vi "FuncVI-MSE.vi"(5 "InstanceRef":T2, 9 "arg list":T1[](array[typedef]) {"num" format="%.2f"}) -> (0 "error out":bool, 3 "result":T1 {"num" format="%.2f"})   [LabVIEW 2021]
doc: "::: CalcExpress Toolkit :::\nCopyright (c) 2000-2026 Konstantin Shifershteyn. All rights reserved."
uses:
  cetypes.llb/CalcExpress Function Argument Info.ctl
  cetypes.llb/CalcExpress Instance RefNum.ctl
  <vilib>/Analysis/NI_AALPro.lvlib
panel:
  in  "max arg num":i32=2
  in  "min arg num":i32=2
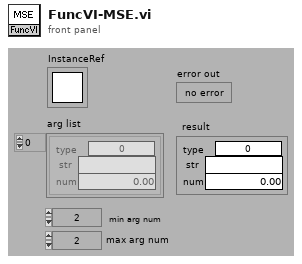
[diagram p1: front panel]
types:
  T1 = typedef "CalcExpress Function Argument Info.ctl" = cluster{"type":u32, "str":string, "num":dbl}
  T2 = typedef "CalcExpress Instance RefNum.ctl" = refnum<k1>
  T3 = enum32{"String", "DBL Number", "identifier", "1D Array of DBL", "2D Array of DBL", "CDB Number", "1D Array of CDB", "2D Array of CDB", "1D Array of String", "2D Array of String", "Unknown data type"}
  T4 = typedef "CalcExpress Data Type.ctl" = enum32{"String", "DBL Number", "identifier", "1D Array of DBL", "2D Array of DBL", "CDB Number", "1D Array of CDB", "2D Array of CDB", "1D Array of String", "2D Array of String", "Unknown data type"}
  T5 = cluster{"use this constant to specify a predefined type":enum32{"String", "DBL Number", "identifier", "1D Array of DBL", "2D Array of DBL", "CDB Number", "1D Array of CDB", "2D Array of CDB", "1D Array of String", "2D Array of String", "Unknown data type"}, string, "mse":dbl}
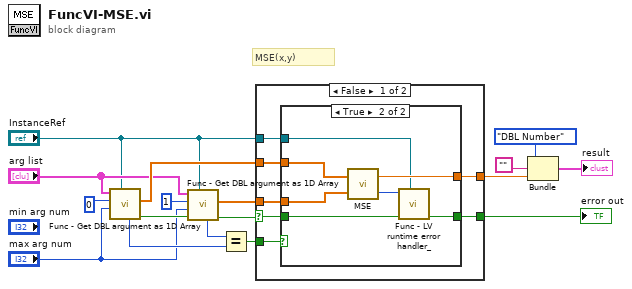
[diagram p0: block diagram]
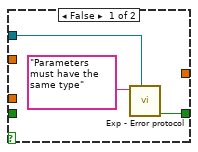
[diagram p2: hidden frame]
diagram:
  # "MSE(x,y)"
  n1 = call "Func - Get DBL argument as 1D Array.vi"("InstanceRef"="InstanceRef", "max arg num"="max arg num", "arg idx"=0, "arg list"="arg list") -> ("error out"=w10:bool, "1D data"=w17:dbl[], "arg type"=w4:T4)  [unwired: 4 in, 1 out]
  n2 = call "Func - Get DBL argument as 1D Array.vi"("InstanceRef"="InstanceRef", "error in"=w10, "max arg num"="max arg num", "arg idx"=1 ("arg index"), "arg list"="arg list") -> ("error out"=w6:bool, "1D data"=w2:dbl[], "arg type"=w5:T4)  [unwired: 3 in, 1 out]
  n3 = Equal?(x=w5, y=w4) -> (x = y?=w3:bool)
  n4 = case shown="False" w6 {
    selector: w6 -> [w23 w35]
    tunnel: w17 -> [w24 _]
    tunnel: [w22 _] -> w14
    tunnel: [w21 w35] -> w15
    tunnel: "InstanceRef" -> [w20 _]
    tunnel: w3 -> [w19 _]
    tunnel: w2 -> [w18 _]
    frame False {
      n5 = case shown="True" w19 {
        tunnel: w24 -> [_ w28]
        tunnel: w23 -> [_ w34]
        tunnel: [_ w32] -> w22
        tunnel: [w27 w31] -> w21
        tunnel: w20 -> [w26 w30]
        tunnel: w18 -> [_ w29]
        frame False {
          n6 = call "Exp - Error protocol.vi"("InstanceRef"=w26, "error message in"="Parameters must have the same type" ("ErrStr")) -> ("error out"=w27:bool)  [unwired: 6 in, 1 out]
        }
        frame True {
          n7 = call <vilib>:"MSE.vi"("X Values"=w29, "Y Values"=w28) -> ("error"=w33:i32, "mse"=w32:dbl)
          n8 = call "Func - LV runtime error handler_.vi"("InstanceRef"=w30, "error in"=w34, "LabVIEW error code"=w33) -> ("error out"=w31:bool)  [unwired: 8 in]
        }
      }
    }
    frame True {
    }
  }
  "error out" <- w15
  n9 = Bundle("use this constant to specify a predefined type"=T3."DBL Number", "", "mse"=w14) -> (→"result":T5)  [unwired: 1 in]
